vi "Beat_Tick.vi"(9 "Last ms":u32, 10 "Beat":i32, 11 "Queue":refnum<queue>) -> (2 "Last ms out":u32, 3 "Beat out":i32)   [LabVIEW 2018]
doc: "Use this template to build a VI to use as a subVI."
panel:
  # "說明：每秒把 D240 放進佇列，值在 1～32767 循環。0 保\n留給「沒有 HMI」。"
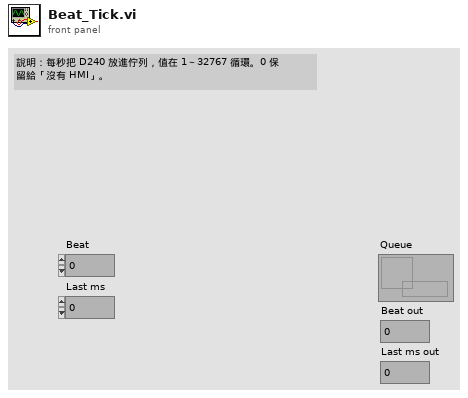
[diagram p1: front panel]
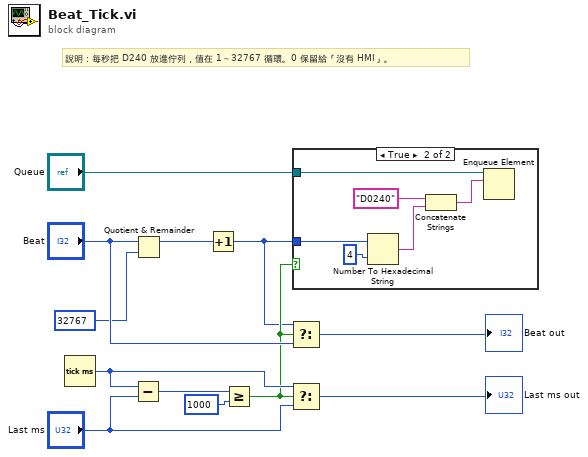
[diagram p0: block diagram]
diagram:
  # "說明：每秒把 D240 放進佇列，值在 1～32767 循環。0 保留給「沒有 HMI」。"
  n1 = Tick Count (ms)() -> (millisecond timer value=w12:u32)
  n2 = Subtract(x=w12, y="Last ms") -> (x-y=w10:u32)
  n3 = Quotient & Remainder(x="Beat", y=32767) -> (x-y*floor(x/y)=w6:i32)  [unwired: 1 out]
  n4 = Increment(x=w6) -> (x+1=w2:i32)
  n5 = Greater Or Equal?(x=w10, y=u32 1000) -> (x >= y?=w5:bool)
  n6 = Select(t=w2, s=w5, f="Beat") -> (s? t:f=→"Beat out":i32)
  n7 = Select(t=w12, s=w5, f="Last ms") -> (s? t:f=→"Last ms out":u32)
  n8 = case shown="True" w5 {
    tunnel: w2 -> [_ w18]
    tunnel: "Queue" -> [_ w14]
    frame False {
    }
    frame True {
      n9 = Number To Hexadecimal String(1:i16 4 ("width (-)"), 2:w18) -> (0:w15:string)
      n10 = Concatenate Strings("D0240", w15) -> (w13:string)
      n11 = Enqueue Element(queue=w14, element=w13) -> ()  [unwired: 2 in, 3 out]
    }
  }
